vi "Synth_Starting_Frequency.vi"(11 "Starting frequency":string) -> ()   [LabVIEW 2024]
uses:
  Serial Port.vi
  <vilib>/Instr/_visa.llb/VISA Configure Serial Port (Instr).vi
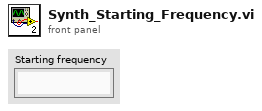
[diagram p1: front panel]
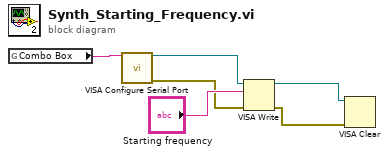
[diagram p0: block diagram]
diagram:
  n1 = global read "Serial Port.vi" "Combo Box"() -> (w1:string)
  n2 = call-poly "VISA Configure Serial Port"("VISA resource name"=w1) -> ("VISA resource name out"=w6:refnum<visa-resource-name>, "error out"=w3:errorcluster)  [unwired: 13 in]
  n3 = VISA Write(VISA resource name=w6, write buffer="Starting frequency", error in (no error)=w3) -> (VISA resource name out=w4:refnum<visa-resource-name>, error out=w2:errorcluster)  [unwired: 1 out]
  n4 = VISA Clear(VISA resource name=w4, error in (no error)=w2) -> ()  [unwired: 2 out]
